vi "Set LED Current.vi"(8 "error in (no error)":errorcluster, 10 "LED Current":dbl, 11 "AS7431 Light Spectrum in":refnum<class "AS7431 11 Ch Light Spectrum Sensor.lvclass">) -> (0 "error out":errorcluster, 3 "AS7431 Light Spectrum out":refnum<class "AS7431 11 Ch Light Spectrum Sensor.lvclass">)   [LabVIEW 2020, in "CTI-Peripheral.lvlib" / "AS7431 11 Ch Light Spectrum Sensor.lvclass"]
uses:
  AS7431 11 Ch Light Spectrum Sensor.lvclass
  AS7431 11 Ch Light Spectrum Sensor.lvclass/AS7431 11 Ch Light Spectrum Sensor.ctl
  CTI/I2C Connection/I2C Connection.lvclass/I2C Connection.ctl
  CTI/Session/I2C Write Data.vi
  CTI/Session/I2C Read Data.vi
  CTI/I2C Connection/I2C Connection.lvclass
panel:
  out "Data":string
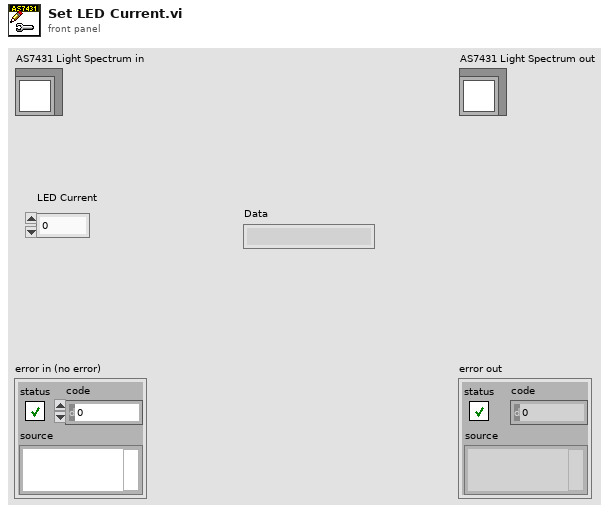
[diagram p1: front panel]
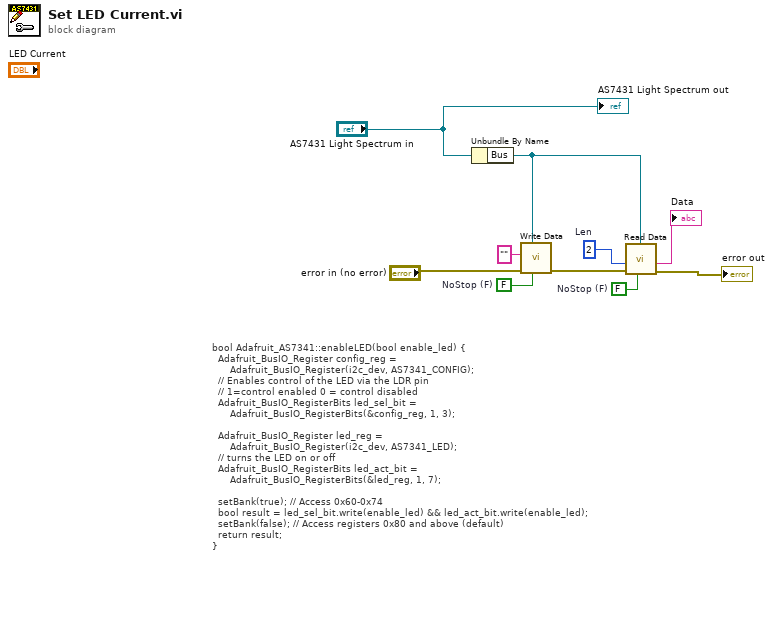
[diagram p0: block diagram]
diagram:
  w7 = FALSE  # NoStop (F)
  w8 = u8 2  # Len
  w9 = FALSE  # NoStop (F)
  # "bool Adafruit_AS7341::enableLED(bool enable_led) {\n  Adafruit_BusIO_Register config_reg =\n      Adafruit_BusIO_Register(i2c_dev, AS7341_CONFIG);\n  // Enables control of the LED via the LDR pin\n  // 1=control enabled 0 = control disabled\n  Adafruit_BusIO_RegisterBits led_sel_bit =\n      Adafruit_BusIO_RegisterBits(&config_reg, 1, 3);\n\n  Adafruit_BusIO_Register led_reg =\n      Adafruit_BusIO_Register(i2c_dev, AS7341_LED);\n  // turns the LED on or off\n  Adafruit_BusIO_RegisterBits led_act_bit =\n      Adafruit_BusIO_RegisterBits(&led_reg, 1, 7);\n\n  setBank(true); // Access 0x60-0x74\n  bool result = led_sel_bit.write(enable_led) && led_act_bit.write(enable_led);\n  setBank(false); // Access registers 0x80 and above (default)\n  return result;\n}"
  n1 = Unbundle By Name("AS7431 Light Spectrum in") -> ("Bus"=w6:refnum<class "I2C Connection.lvclass">)
  n2 = call "Write Data.vi"("NoStop (F)"=w9, "I2C Connection"=w6, "error in (no error)"="error in (no error)", "Data"="") -> ("error out"=w5:errorcluster)  [unwired: 7 in]
  n3 = call "Read Data.vi"("NoStop (F)"=w7, "I2C Connection"=w6, "error in (no error)"=w5, "Len"=w8) -> ("error out"=→"error out":errorcluster, "Data"=→"Data":string)  [unwired: 6 in]
  "AS7431 Light Spectrum out" <- "AS7431 Light Spectrum in"
